vi "Sound_Bank_Load.vi"(11 "error in":errorcluster) -> (4 "Bank":cluster{"Y":dbl[]}[](array[cluster]), 15 "error out":errorcluster)   [LabVIEW 2020, in "GH_Audio.lvlib"]
doc: "Loads all sound effects once (order = priority: gameover, death, treasure, level, life, torch, door, key, hoard, coin, ready, jump, slide, then the music): Resources\\Sounds\\<name>.wav, first channel as samples (-1..1)."
uses:
  GH_Audio.lvlib
  Level/GH_Level.lvlib
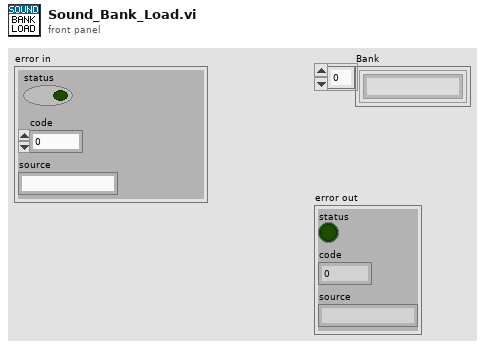
[diagram p1: front panel]
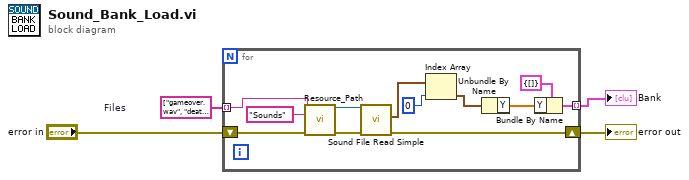
[diagram p0: block diagram]
diagram:
  w2 = string[] ["gameover.wav", "death.wav", "treasure.wav", "level.wav", "life.wav", "torch.wav", "door.wav", "key.wav", "hoard.wav", "coin.wav", "ready.wav", "jump.wav", "slide.wav", "music.wav"]  # Files
  n1 = for {
    tunnel: w2 -> [w5] mode=indexing
    shift-right: [w7] -> w3
    shift-left: "error in" -> [w6]
    tunnel: [w16] -> w4 mode=indexing
    n2 = call "Resource_Path.vi"("File name"=w5, "Subfolder"="Sounds", "error in"=w6) -> ("Path"=w9:path, "error out"=w10:errorcluster)  [unwired: 11 in]
    n3 = call <vilib>:"Sound File Read Simple.vi"("error in (no error)"=w10, "path"=w9) -> ("error out"=w7:errorcluster, "data"=w11:waveform(dbl)[])  [unwired: 6 in, 2 out]
    n4 = Index Array(array=w11, index=0) -> (element=w13:waveform(dbl))
    n5 = Unbundle By Name(w13) -> ("Y"=w14:dbl[])
    n6 = Bundle By Name(cluster=cluster{"Y":dbl[]} {"Y"=[]}, "Y"=w14) -> (w16:cluster{"Y":dbl[]})
  }
  "Bank" <- w4
  "error out" <- w3
